vi "CSMKVMap-Write.vi"(5 "name":string, 6 "Error in":errorcluster caption="Error in (no error)", 9 "value":variant) -> (0 "Error out":errorcluster)   [LabVIEW 2017, in "Communicable State Machine.lvlib"]
uses:
  Communicable State Machine.lvlib
  ChangeFlag/ChangeFlag-Write.vi
  Utility/Random Change Flag.vi
  ChangeFlag/ChangeFlagDB.vi
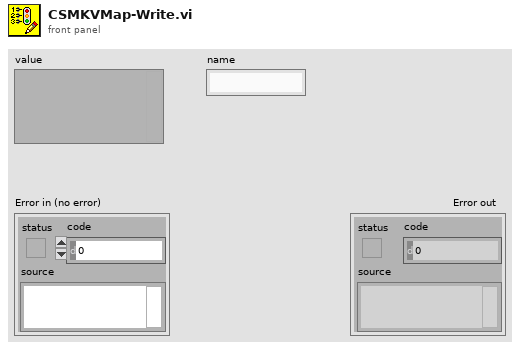
[diagram p1: front panel]
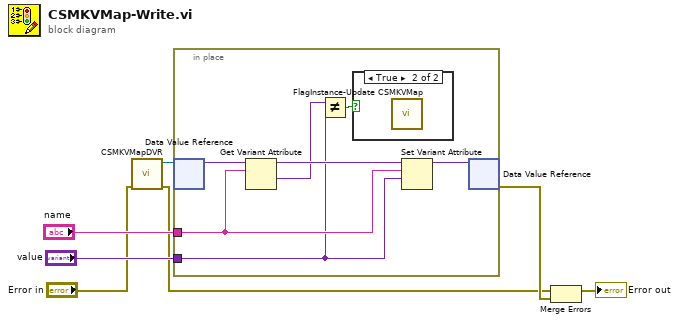
[diagram p0: block diagram]
diagram:
  n1 = call "CSMKVMapDVR.vi"("error in (no error)"="Error in") -> ("error out"=w1:errorcluster, "KVMapDVR"=w3:refnum<data-value>)  [unwired: 9 in]
  n2 = in-place {
    in-place-border: "name" -> [w10]
    in-place-border: "value" -> [w9]
    n3 = in-place-dvr #1(w3) -> (w14:variant)  [unwired: 1 out]
    n4 = Get Variant Attribute(Variant=w14, name=w10) -> (duplicate Variant=w12:variant, value=w11:variant)  [unwired: 2 in, 2 out]
    n5 = Not Equal?(x=w11, y=w9) -> (x != y?=w8:bool)
    n6 = case shown="True" w8 {
      frame False {
      }
      frame True {
        n7 = call "FlagInstance-Update CSMKVMap.vi"() -> ()  [unwired: 10 in, 2 out]
      }
    }
    n8 = Set Variant Attribute(Variant=w12, name=w10, value=w9) -> (Variant out=w13:variant)  [unwired: 1 in, 2 out]
    n9 = in-place-dvr #1(w13) -> (w5:errorcluster)  [unwired: 1 out]
  }
  n10 = Merge Errors(w1, w5) -> (→"Error out":errorcluster)
